vi "Send Exit Message to All MHLs.vi"(8 "error in (no error)":errorcluster, 11 "Message Queues":T1) -> (0 "error out":errorcluster)   [LabVIEW 2026, in "UI.lvlib"]
doc: "すべてのメッセージキューにExitメッセージを送る。"
uses:
  UI.lvlib
  support/Message Queue/All Message Queues.ctl
  support/Message Queue/Message Cluster.ctl
  e7f3e565-3e0e-48e1-9954-56ed745e6014.vi
  e7f3e565-3e0e-48e1-9954-56ed745e6014.vi/904feb24-0ee5-4d46-a973-81b984403c80.vi
  support/Message Queue/Enqueue Message (Single).vi
  support/Message Queue/Message Queue.lvlib
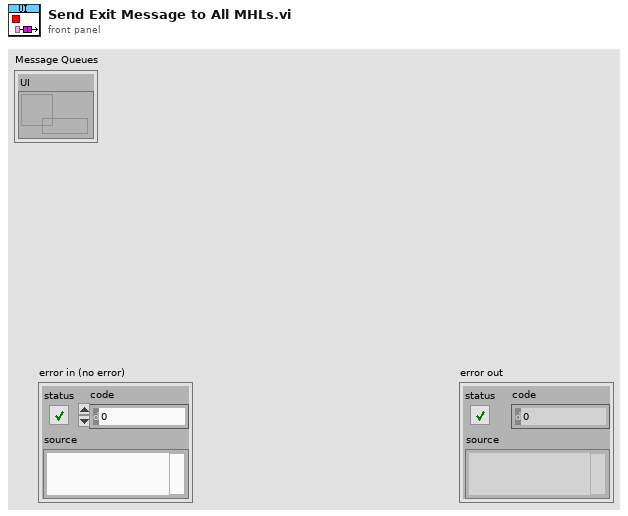
[diagram p1: front panel]
types:
  T1 = typedef "Message Queue.lvlib/All Message Queues.ctl" = cluster{"UI":refnum<queue>}
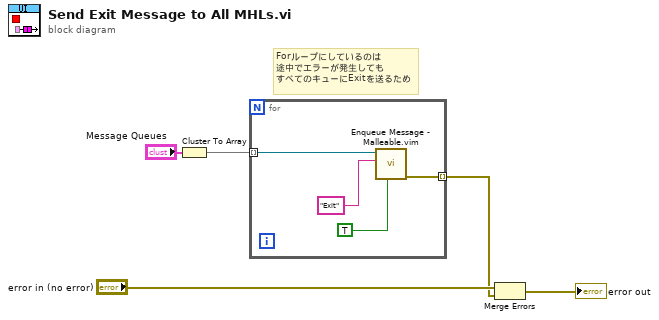
[diagram p0: block diagram]
diagram:
  # "Forループにしているのは\n途中でエラーが発生しても\nすべてのキューにExitを送るため"
  n1 = Cluster To Array(cluster="Message Queues") -> (array=w4:refnum<queue>[])
  n2 = for {
    tunnel: w4 -> [w7] mode=indexing
    tunnel: [w6] -> w1 mode=indexing
    n3 = call "Enqueue Message - Malleable.vim"("Priority Message? (F)"=TRUE, "Message"="Exit", "Message Queue"=w7) -> ("error out"=w6:errorcluster)  [unwired: 7 in, 1 out]
  }
  n4 = Merge Errors("error in (no error)", w1) -> (→"error out":errorcluster)
